vi "Scan Engine Initialization VI.vi"(8 "error in (no error)":errorcluster, 10 "Custom XML":string, 11 "Device Item Ref in":T1 format="%.0x") -> (0 "error out":errorcluster, 3 "Device Item Ref out":T1 format="%.0x")   [LabVIEW 2020, in "SEECD System Explorer.lvlib"]
uses:
  SEECD System Explorer.lvlib
  <vilib>/NI VeriStand/Custom Device API/Custom Device Item Ref.ctl
  <vilib>/NI VeriStand/Custom Device API/Custom Device Channel.ctl
  <vilib>/NI VeriStand/Custom Device API/Custom Device Channel Type.ctl
  Shared/Globals/Property Strings.vi
  <vilib>/NI VeriStand/Custom Device API/Set Item Property (U16).vi
  <vilib>/NI VeriStand/Custom Device API/Custom Device API.lvlib
  Shared/SEECD Shared.lvlib
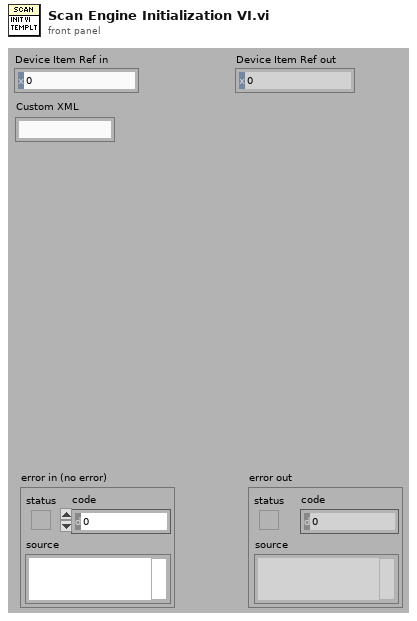
[diagram p1: front panel]
types:
  T1 = typedef "Custom Device API.lvlib/Custom Device Item Ref.ctl" = u64
  T2 = typedef "Custom Device API.lvlib/Custom Device Channel.ctl" = cluster{"Type":T3, "Units":string, "Default Value":dbl, "Faultable":bool, "Scalable":bool}
  T3 = typedef "Custom Device API.lvlib/Custom Device Channel Type.ctl" = enum16{"Input", "Output"}
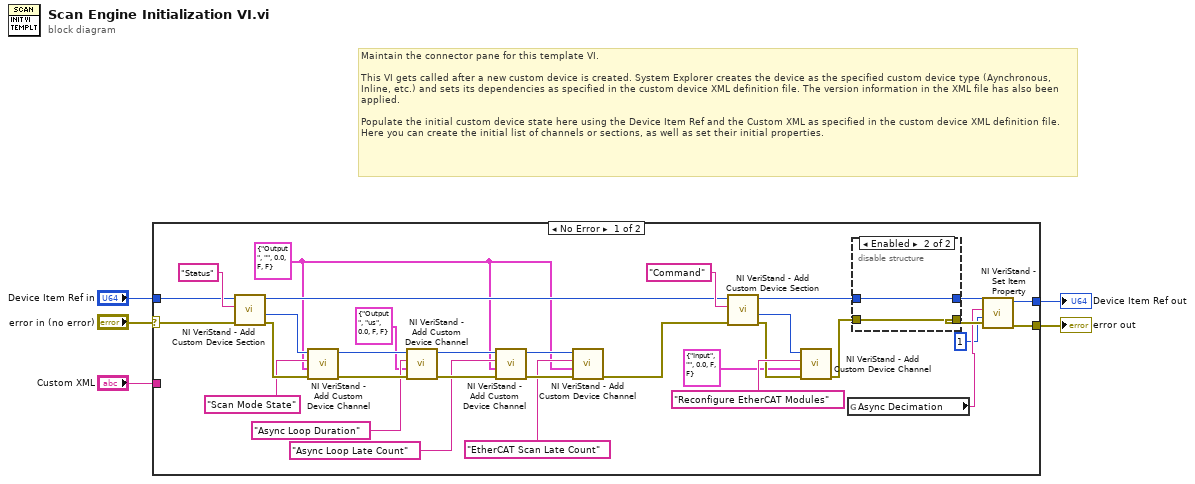
[diagram p0: block diagram]
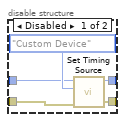
[diagram p2: hidden frame]
diagram:
  # "Maintain the connector pane for this template VI.\n\nThis VI gets called after a new custom device is created. System Explorer creates the device as the specified custom device type (Aynchronous, Inline, etc.) and sets its dependencies as specified in the custom device XML definition file. The version information in the XML file has also been applied.\n\nPopulate the initial custom device state here using the Device Item Ref and the Custom XML as specified in the custom device XML definition file. Here you can create the initial list of channels or sections, as well as set their initial properties."
  n1 = case shown="No Error" "error in (no error)" {
    selector: "error in (no error)" -> [w18 w46]
    tunnel: [w23 w46] -> w5
    tunnel: [w22 w45] -> w3
    tunnel: "Device Item Ref in" -> [w19 w45]
    tunnel: "Custom XML" -> [_ _]
    frame No Error {
      w6 = T2 {"Type"=enum."Output", "Units"="", "Default Value"=0.0, "Faultable"=FALSE, "Scalable"=FALSE} ("Channel")
      n2 = call <vilib>:"NI VeriStand - Add Custom Device Section.vi"("error in (no error)"=w18, "Section Name"="Status", "Parent Ref in"=w19) -> ("error out"=w35:errorcluster, "Section Ptr"=w36:T1, "Parent Ref out"=w28:T1)  [unwired: 5 in, 1 out]
      n3 = call <vilib>:"NI VeriStand - Add Custom Device Channel.vi"("error in (no error)"=w35, "Channel"=w6, "Channel Name"="Scan Mode State", "Parent Ref in"=w36) -> ("error out"=w17:errorcluster, "Parent Ref out"=w14:T1)  [unwired: 4 in, 2 out]
      n4 = call <vilib>:"NI VeriStand - Add Custom Device Channel.vi"("error in (no error)"=w17, "Channel"=T2 {"Type"=enum."Output", "Units"="us", "Default Value"=0.0, "Faultable"=FALSE, "Scalable"=FALSE}, "Channel Name"="Async Loop Duration", "Parent Ref in"=w14) -> ("error out"=w16:errorcluster, "Parent Ref out"=w15:T1)  [unwired: 4 in, 2 out]
      n5 = call <vilib>:"NI VeriStand - Add Custom Device Channel.vi"("error in (no error)"=w16, "Channel"=w6, "Channel Name"="Async Loop Late Count", "Parent Ref in"=w15) -> ("error out"=w10:errorcluster, "Parent Ref out"=w11:T1)  [unwired: 4 in, 2 out]
      n6 = call <vilib>:"NI VeriStand - Add Custom Device Channel.vi"("error in (no error)"=w10, "Channel"=w6, "Channel Name"="EtherCAT Scan Late Count", "Parent Ref in"=w11) -> ("error out"=w8:errorcluster)  [unwired: 4 in, 3 out]
      n7 = call <vilib>:"NI VeriStand - Add Custom Device Section.vi"("error in (no error)"=w8, "Section Name"="Command", "Parent Ref in"=w28) -> ("error out"=w32:errorcluster, "Section Ptr"=w31:T1, "Parent Ref out"=w27:T1)  [unwired: 5 in, 1 out]
      n8 = call <vilib>:"NI VeriStand - Add Custom Device Channel.vi"("error in (no error)"=w32, "Channel"=T2 {"Type"=enum."Input", "Units"="", "Default Value"=0.0, "Faultable"=FALSE, "Scalable"=FALSE}, "Channel Name"="Reconfigure EtherCAT Modules", "Parent Ref in"=w31) -> ("error out"=w26:errorcluster)  [unwired: 4 in, 3 out]
      n9 = global read "Property Strings.vi" "Async Decimation"() -> (w21:string)
      n10 = disable-structure shown="Enabled" {
        disable-tunnel: w27 -> [w41 w44]
        disable-tunnel: w26 -> [w40 w43]
        disable-tunnel: [w39 w44] -> w25
        disable-tunnel: [w38 w43] -> w24
        frame Disabled {
          n11 = call "Set Timing Source.vi"("error in (no error)"=w40, "Timing Source"=enum16{"Automatic", "Custom Device"}."Custom Device", "Item Ref in"=w41) -> ("error out"=w38:errorcluster, "Item Ref out"=w39:T1)  [unwired: 7 in]
        }
        frame Enabled {
        }
      }
      n12 = call-poly <vilib>:"NI VeriStand - Set Item Property.vi"("error in (no error)"=w24, "Value"=u16 1, "Property Name"=w21, "Item Ref in"=w25) -> ("error out"=w23:errorcluster, "Item Ref out"=w22:T1)  [unwired: 5 in, 1 out]
    }
    frame Error {
    }
  }
  "error out" <- w5
  "Device Item Ref out" <- w3
